vi "Write Main Config.vi"(8 "error in (no error)":errorcluster, 9 "Config":string, 10 "Main Config Path":path, 11 "System Config Module in":refnum<class "System Config Module.lvclass">) -> (0 "error out":errorcluster, 3 "System Config Module out":refnum<class "System Config Module.lvclass">)   [LabVIEW 2020, in "Volatus.lvlib" / "System Config Module.lvclass"]
uses:
  System Config Module.lvclass
  System Config Module.lvclass/System Config Module.ctl
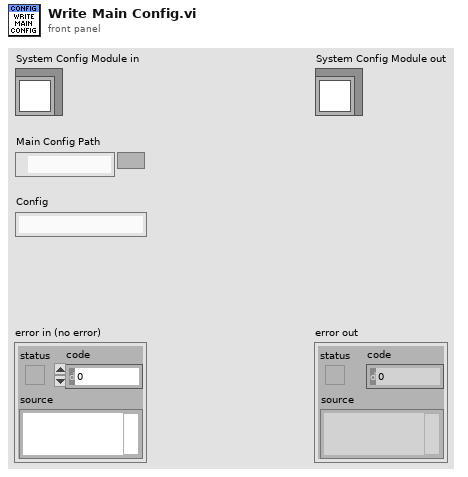
[diagram p1: front panel]
types:
  T1 = enum16{"open", "replace", "create", "open or create", "replace or create", "replace or create with confirmation"}
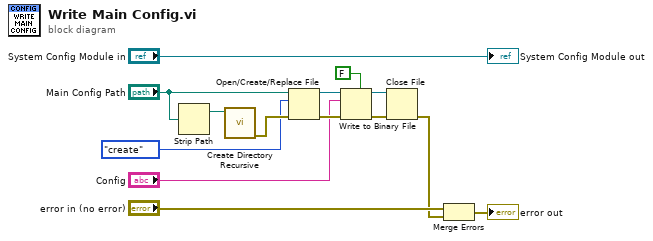
[diagram p0: block diagram]
diagram:
  n1 = Strip Path(path="Main Config Path") -> (stripped path=w1:path)  [unwired: 1 out]
  n2 = call <vilib>:"Create Directory Recursive.vi"("directory"=w1) -> ("error out"=w14:errorcluster)  [unwired: 4 in, 2 out]
  n3 = Open/Create/Replace File(file path (use dialog)="Main Config Path", error in=w14, operation (0:open)=T1."create") -> (refnum out=w10:refnum<file>, error out=w9:errorcluster)  [unwired: 3 in, 1 out]
  n4 = Write to Binary File(file (use dialog)=w10, data="Config", error in=w9, 5:FALSE ("prepend array or string size? (T)")) -> (refnum out=w5:refnum<file>, error out=w6:errorcluster)  [unwired: 2 in, 1 out]
  n5 = Close File(refnum=w5, error in=w6) -> (error out=w3:errorcluster)  [unwired: 1 out]
  n6 = Merge Errors("error in (no error)", w3) -> (→"error out":errorcluster)
  "System Config Module out" <- "System Config Module in"
